vi "LabVIEW.Service.Convert_a_list_of_API_Tokens_from_JSON_to_Tabel.vi"(8 "error in (no error)":errorcluster caption="Fehler (Eingang, kein Fehler)", 11 "Body":string) -> (0 "error out":errorcluster caption="Fehler (Ausgang)", 3 "API Tokens":string[][](array[string]))   [LabVIEW 2019]
uses:
  <vilib>/JDP Science/JSONtext/String Subset.vi
  <vilib>/JDP Science/JSONtext/support/Strip Quotes and Unescape.vi
  <vilib>/JDP Science/JSONtext/support/Unescape JSON string.vi
  <vilib>/JDP Science/JSONtext/Parsing/Parse Full Path or Item Name.vi
  <vilib>/JDP Science/JSONtext/Offset/Find Item Locations by Path.vi
  <vilib>/JDP Science/JSONtext/JSONtext.lvlib
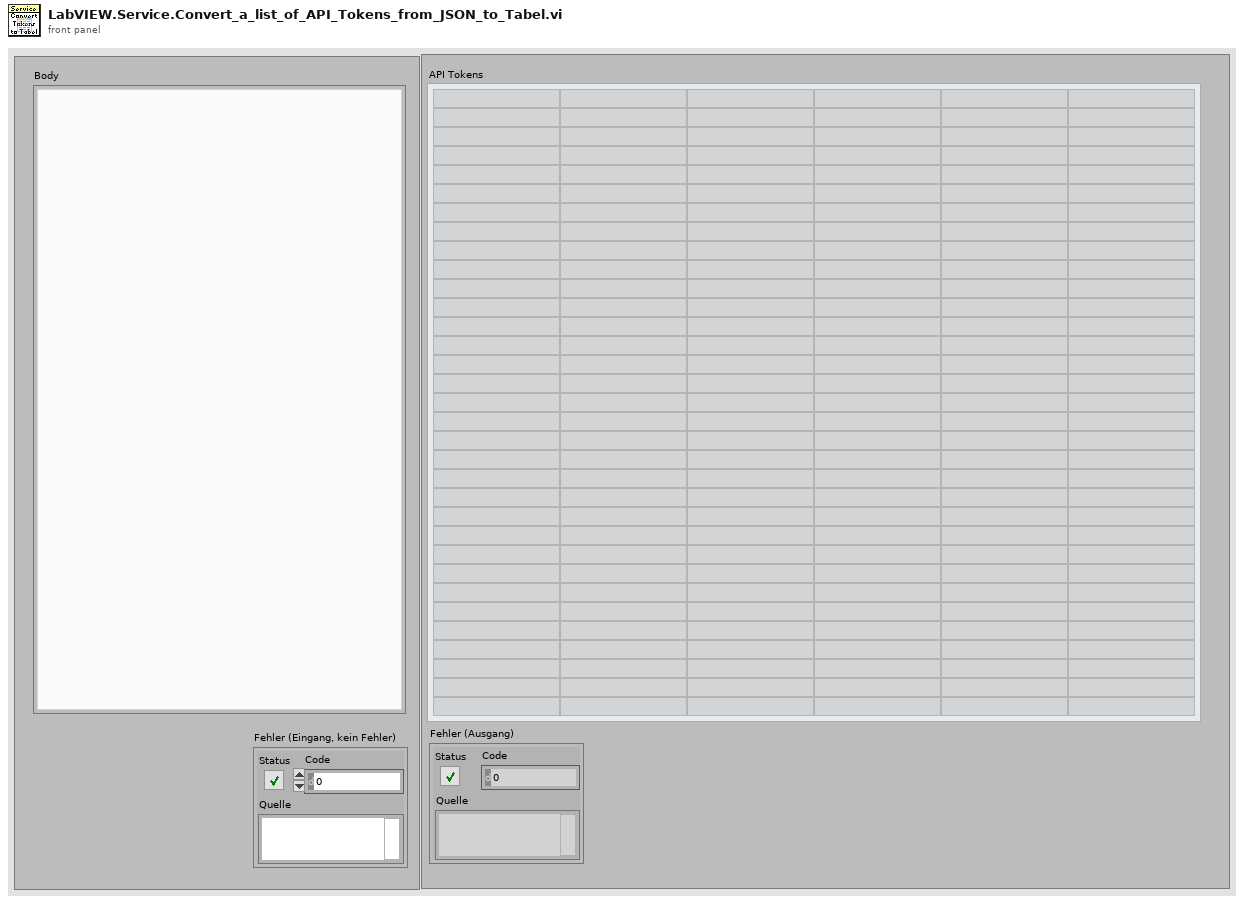
[diagram p1: front panel]
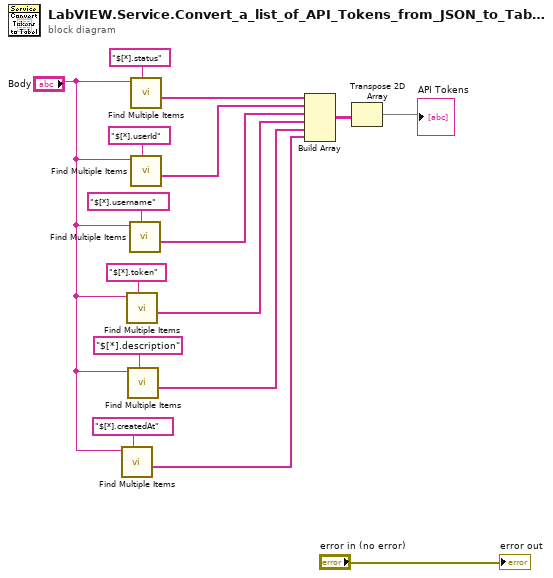
[diagram p0: block diagram]
diagram:
  n1 = call <vilib>:"Find Multiple Items.vi"("$Path or Item Name"="$[*].createdAt", "JSON"="Body") -> ("<JSON>"=w4:string[])  [unwired: 6 in, 3 out]
  n2 = call <vilib>:"Find Multiple Items.vi"("$Path or Item Name"="$[*].token", "JSON"="Body") -> ("<JSON>"=w6:string[])  [unwired: 6 in, 3 out]
  n3 = call <vilib>:"Find Multiple Items.vi"("$Path or Item Name"="$[*].description", "JSON"="Body") -> ("<JSON>"=w5:string[])  [unwired: 6 in, 3 out]
  n4 = call <vilib>:"Find Multiple Items.vi"("$Path or Item Name"="$[*].username", "JSON"="Body") -> ("<JSON>"=w7:string[])  [unwired: 6 in, 3 out]
  n5 = call <vilib>:"Find Multiple Items.vi"("$Path or Item Name"="$[*].status", "JSON"="Body") -> ("<JSON>"=w9:string[])  [unwired: 6 in, 3 out]
  n6 = call <vilib>:"Find Multiple Items.vi"("$Path or Item Name"="$[*].userId", "JSON"="Body") -> ("<JSON>"=w8:string[])  [unwired: 6 in, 3 out]
  n7 = Build Array(w9, w8, w7, w6, w5, w4) -> (w3:string[][])
  n8 = Transpose 2D Array(2D array=w3) -> (transposed array=→"API Tokens":string[][])
  "error out" <- "error in (no error)"
